vi "ASD Threshold Function VI.vi"(8 "D thred (pA)":dbl, 9 "U thred (pA)":dbl, 11 "Estimated BL":dbl[](array[numeric])) -> (2 "Down Thre Func":dbl[](array[numeric]), 3 "UP Thre Func":dbl[](array[numeric]))   [LabVIEW 2018]
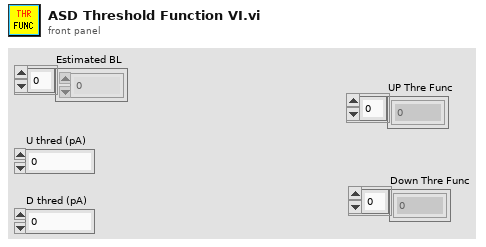
[diagram p1: front panel]
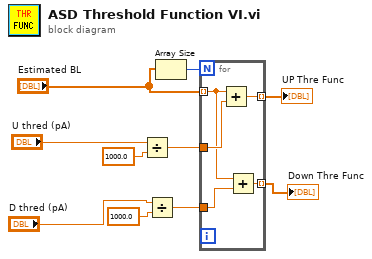
[diagram p0: block diagram]
diagram:
  n1 = Divide(x="U thred (pA)", y=1000.0) -> (x/y=w8:dbl)
  n2 = Divide(x="D thred (pA)", y=1000.0) -> (x/y=w2:dbl)
  n3 = Array Size(array="Estimated BL") -> (size(s)=w10:i32)
  n4 = for {
    N: w10 -> [_]
    tunnel: "Estimated BL" -> [w13] mode=indexing
    tunnel: w8 -> [w15]
    tunnel: [w14] -> w6 mode=indexing
    tunnel: w2 -> [w12]
    tunnel: [w11] -> w1 mode=indexing
    n5 = Add(x=w13, y=w15) -> (x+y=w14:dbl)
    n6 = Add(x=w13, y=w12) -> (x+y=w11:dbl)
  }
  "UP Thre Func" <- w6
  "Down Thre Func" <- w1
